vi "Generation.vi"() -> (2 "Phone Numbers":string[][](array[string]))   [LabVIEW 2021]
uses:
  <vilib>/numeric/Random Number (Range) U64.vi
  <vilib>/numeric/sub_Random U32.vi
panel:
  in  "ALLER":bool
  in  "N_I":i8
  in  "N_M":i8
  in  "N_SOO":i8
  in  "N_SE":i8
  in  "N_NE":i8
  in  "N_NO":i8
  in  "N_IDF":i8
  # "Combien de fois chaque\n numéro doit être\n généré"
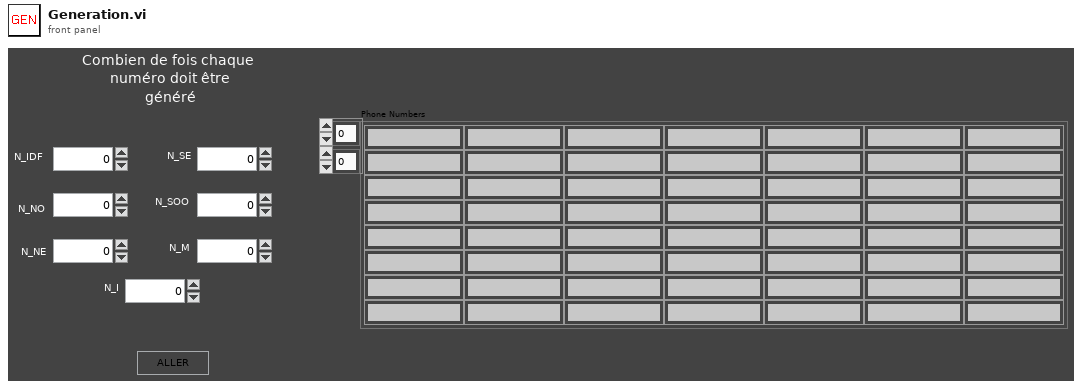
[diagram p1: front panel]
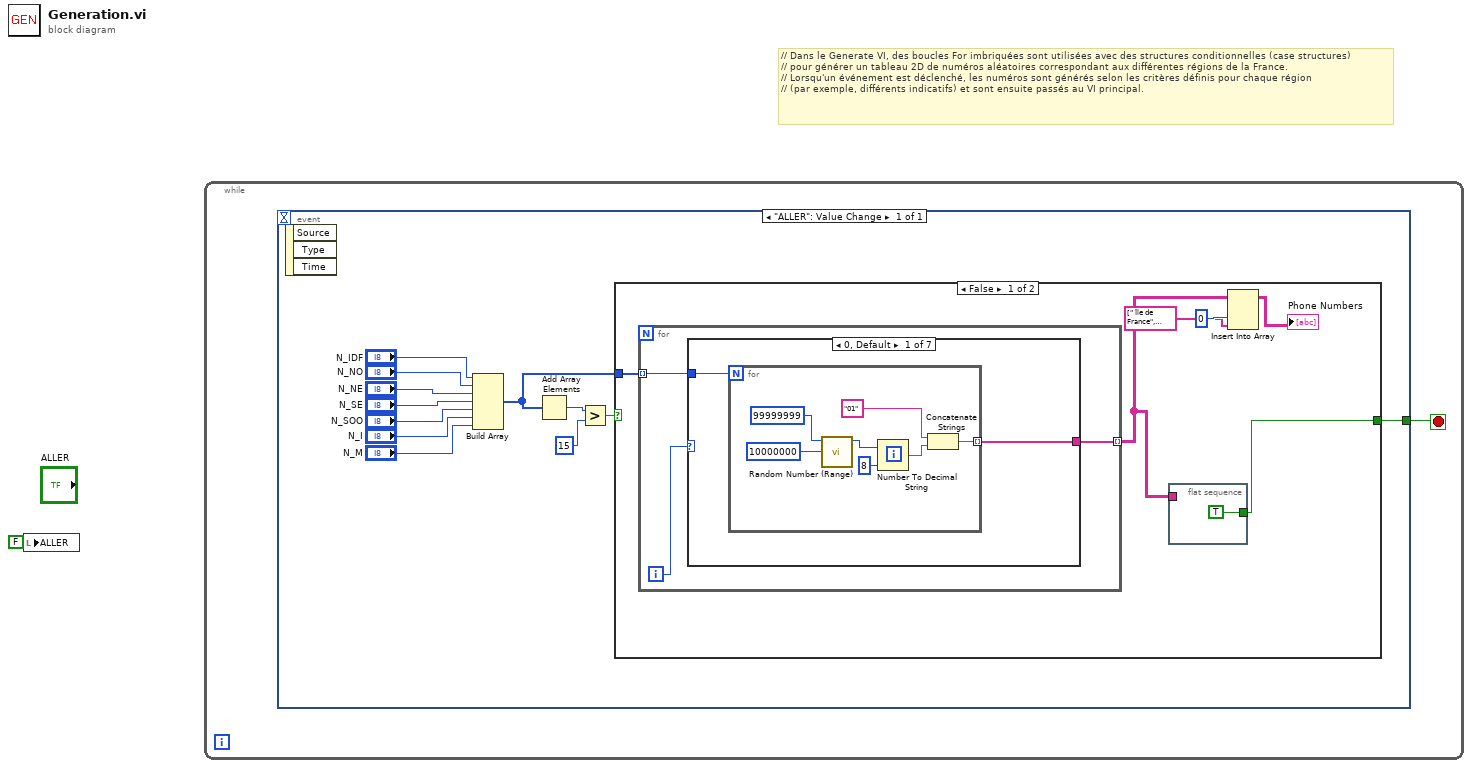
[diagram p0: block diagram]
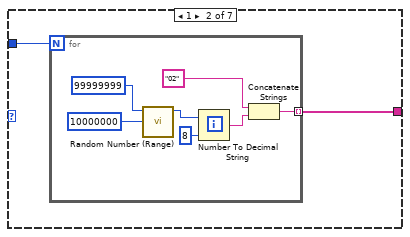
[diagram p2: hidden frame]
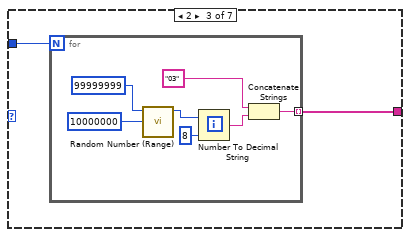
[diagram p3: hidden frame]
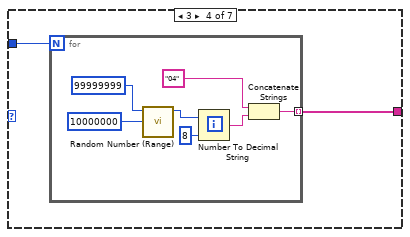
[diagram p4: hidden frame]
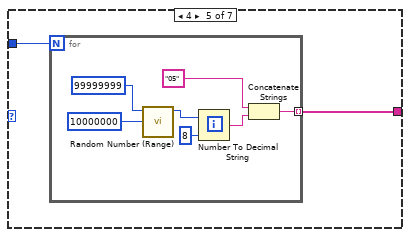
[diagram p5: hidden frame]
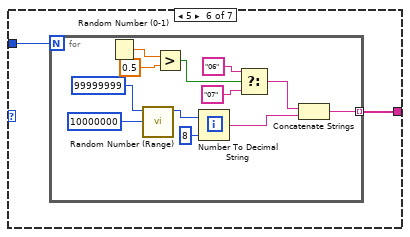
[diagram p6: hidden frame]
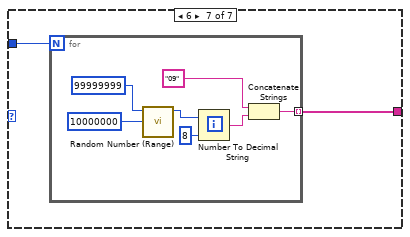
[diagram p7: hidden frame]
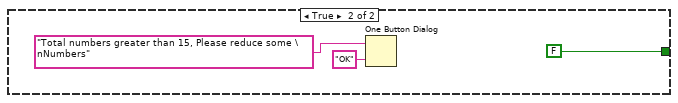
[diagram p8: hidden frame]
diagram:
  # "// Dans le Generate VI, des boucles For imbriquées sont utilisées avec des structures conditionnelles (case structures)\n// pour générer un tableau 2D de numéros aléatoires correspondant aux différentes régions de la France.\n// Lorsqu'un événement est déclenché, les numéros sont générés selon les critères définis pour chaque région\n// (par exemple, différents indicatifs) et sont ensuite passés au VI principal."
  n1 = local write "ALLER"(FALSE ("Fill")) -> ()
  n2 = while {
    stop <- w2 stop-if-true
    n3 = event shown="[0] \"ALLER\": Value Change" {
      selector: _ -> [_]
      dyn-events: _ -> [_]
      timeout: _ -> [_]
      tunnel: [w11] -> w2
      event "ALLER": Value Change {
        n4 = event-data() -> ()  [unwired: 1 in, 3 out]
        n5 = Build Array("N_IDF", "N_NO", "N_NE", "N_SE", "N_SOO", "N_I", "N_M") -> (w3:i8[])
        n6 = Add Array Elements(numeric array=w3) -> (sum=w14:i8)
        n7 = Greater?(x=w14, y=i8 15) -> (0:w12:bool)
        n8 = case shown="False" w12 {
          tunnel: w3 -> [w20 _]
          tunnel: [w19 FALSE] -> w11
          frame False {
            n9 = for {
              tunnel: w20 -> [w24] mode=indexing
              tunnel: [w23] -> w18 mode=indexing
              i -> [w22]
              n10 = case shown="0, Default" w22 {
                tunnel: w24 -> [w26 w35 w44 w53 w62 w71 w85]
                tunnel: [w25 w34 w43 w52 w61 w70 w84] -> w23
                frame 0, Default {
                  n11 = for {
                    N: w26 -> [_]
                    tunnel: [w33] -> w25 mode=indexing
                    n12 = call-poly <vilib>:"Random Number (Range).vi"("lower bound (0)"=u64 10000000 ("upper bound (100)"), "upper bound (100)"=u64 99999999 ("lower bound (0)")) -> ("number"=w32:u64)  [unwired: 9 in]
                    n13 = Number To Decimal String(number=w32, width (-)=i16 8) -> (decimal integer string=w30:string)
                    n14 = Concatenate Strings("01", w30) -> (w33:string)
                  }
                }
                frame 1 {
                  n15 = for {
                    N: w35 -> [_]
                    tunnel: [w42] -> w34 mode=indexing
                    n16 = call-poly <vilib>:"Random Number (Range).vi"("lower bound (0)"=u64 10000000 ("upper bound (100)"), "upper bound (100)"=u64 99999999 ("lower bound (0)")) -> ("number"=w41:u64)  [unwired: 9 in]
                    n17 = Number To Decimal String(number=w41, width (-)=i16 8) -> (decimal integer string=w39:string)
                    n18 = Concatenate Strings("02", w39) -> (w42:string)
                  }
                }
                frame 2 {
                  n19 = for {
                    N: w44 -> [_]
                    tunnel: [w51] -> w43 mode=indexing
                    n20 = call-poly <vilib>:"Random Number (Range).vi"("lower bound (0)"=u64 10000000 ("upper bound (100)"), "upper bound (100)"=u64 99999999 ("lower bound (0)")) -> ("number"=w50:u64)  [unwired: 9 in]
                    n21 = Number To Decimal String(number=w50, width (-)=i16 8) -> (decimal integer string=w48:string)
                    n22 = Concatenate Strings("03", w48) -> (w51:string)
                  }
                }
                frame 3 {
                  n23 = for {
                    N: w53 -> [_]
                    tunnel: [w60] -> w52 mode=indexing
                    n24 = call-poly <vilib>:"Random Number (Range).vi"("lower bound (0)"=u64 10000000 ("upper bound (100)"), "upper bound (100)"=u64 99999999 ("lower bound (0)")) -> ("number"=w59:u64)  [unwired: 9 in]
                    n25 = Number To Decimal String(number=w59, width (-)=i16 8) -> (decimal integer string=w57:string)
                    n26 = Concatenate Strings("04", w57) -> (w60:string)
                  }
                }
                frame 4 {
                  n27 = for {
                    N: w62 -> [_]
                    tunnel: [w69] -> w61 mode=indexing
                    n28 = call-poly <vilib>:"Random Number (Range).vi"("lower bound (0)"=u64 10000000 ("upper bound (100)"), "upper bound (100)"=u64 99999999 ("lower bound (0)")) -> ("number"=w68:u64)  [unwired: 9 in]
                    n29 = Number To Decimal String(number=w68, width (-)=i16 8) -> (decimal integer string=w66:string)
                    n30 = Concatenate Strings("05", w66) -> (w69:string)
                  }
                }
                frame 5 {
                  n31 = for {
                    N: w71 -> [_]
                    tunnel: [w83] -> w70 mode=indexing
                    n32 = Random Number (0-1)() -> (number: 0 to 1=w77:dbl)
                    n33 = call-poly <vilib>:"Random Number (Range).vi"("lower bound (0)"=u64 10000000 ("upper bound (100)"), "upper bound (100)"=u64 99999999 ("lower bound (0)")) -> ("number"=w82:u64)  [unwired: 9 in]
                    n34 = Greater?(x=w77, y=0.5) -> (0:w74:bool)
                    n35 = Number To Decimal String(number=w82, width (-)=i16 8) -> (decimal integer string=w80:string)
                    n36 = Select(t="06", s=w74, f="07") -> (s? t:f=w72:string)
                    n37 = Concatenate Strings(w72, w80) -> (w83:string)
                  }
                }
                frame 6 {
                  n38 = for {
                    N: w85 -> [_]
                    tunnel: [w92] -> w84 mode=indexing
                    n39 = call-poly <vilib>:"Random Number (Range).vi"("lower bound (0)"=u64 10000000 ("upper bound (100)"), "upper bound (100)"=u64 99999999 ("lower bound (0)")) -> ("number"=w91:u64)  [unwired: 9 in]
                    n40 = Number To Decimal String(number=w91, width (-)=i16 8) -> (decimal integer string=w89:string)
                    n41 = Concatenate Strings("09", w89) -> (w92:string)
                  }
                }
              }
            }
            n42 = flat-sequence {
              tunnel: w18 -> [_]
              tunnel: [TRUE] -> w19
              frame #0 {
              }
            }
            n43 = Insert Into Array(array=w18, index (col)=0 ("disabled index (col)"), new element=string[] [" Île de France", "Nord Ouest", "Nord Est", " Sud Est", "Sud Ouest-Outremer", "mobiles particuliers ", "internet particuliers"] ("new element/subarray")) -> (→"Phone Numbers":string[][])  [unwired: 1 in]
          }
          frame True {
            n44 = One Button Dialog(message="Total numbers greater than 15, Please reduce some \nNumbers", button name ("OK")="OK") -> ()  [unwired: 1 out]
          }
        }
      }
    }
  }
